vi "TDMS_M1509 (SubVI).vi"(0 "참조 번호 입력":refnum<k34>, 5 "Value":dbl[](array[numeric]), 7 "Value 3":dbl[](array[numeric]), 9 "Value 2":dbl[](array[numeric]), 11 "에러 입력(에러 없음)":errorcluster) -> (4 "참조 번호 출력":refnum<k34>, 15 "에러 출력":errorcluster)   [LabVIEW 2019]
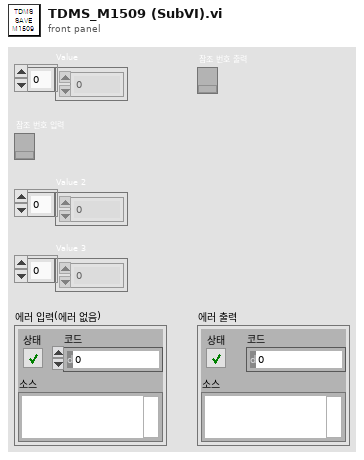
[diagram p1: front panel]
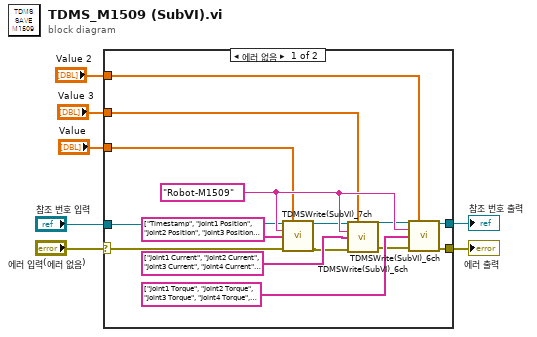
[diagram p0: block diagram]
diagram:
  n1 = case shown="에러 없음" "에러 입력(에러 없음)" {
    selector: "에러 입력(에러 없음)" -> [w8 w24]
    tunnel: [w22 w24] -> w7
    tunnel: [w21 w23] -> w6
    tunnel: "참조 번호 입력" -> [w16 w23]
    tunnel: "Value 2" -> [w11 _]
    tunnel: "Value 3" -> [w10 _]
    tunnel: "Value" -> [w9 _]
    frame No Error {
      w18 = "Robot-M1509" ("그룹입력")
      n2 = call "TDMSWrite(SubVI)_7ch.vi"("tdms file out 입력"=w16, "배열"=w9, "그룹입력"=w18, "채널입력"=string[] ["Timestamp", "Joint1 Position", "Joint2 Position", "Joint3 Position", "Joint4 Position", "Joint5 Position", "Joint6 Position"], "에러 입력"=w8) -> ("참조 번호 출력"=w14:refnum<k34>, "에러 출력"=w15:errorcluster)  [unwired: 9 in]
      n3 = call "TDMSWrite(SubVI)_6ch.vi"("tdms file out 입력"=w14, "배열"=w10, "그룹입력"=w18, "채널입력"=string[] ["Joint1 Current", "Joint2 Current", "Joint3 Current", "Joint4 Current", "Joint5 Current", "Joint6 Current"], "에러 입력"=w15) -> ("참조 번호 출력"=w13:refnum<k34>, "에러 출력"=w12:errorcluster)  [unwired: 9 in]
      n4 = call "TDMSWrite(SubVI)_6ch.vi"("tdms file out 입력"=w13, "배열"=w11, "그룹입력"=w18, "채널입력"=string[] ["Joint1 Torque", "Joint2 Torque", "Joint3 Torque", "Joint4 Torque", "Joint5 Torque", "Joint6 Torque"], "에러 입력"=w12) -> ("참조 번호 출력"=w21:refnum<k34>, "에러 출력"=w22:errorcluster)  [unwired: 9 in]
    }
    frame Error {
    }
  }
  "에러 출력" <- w7
  "참조 번호 출력" <- w6
